vi "RemoteVI Landing Server.vi"(0 "VI":refnum<vi>, 1 "share":T1, 5 "port":u16=8088, 7 "fps":dbl=20.0, 9 "stop notifier name":string, 11 "error in":errorcluster) -> (15 "error out":errorcluster)   [LabVIEW 2020, in "RemoteVI.lvlib"]
doc: "RemoteVI Server's landing page: a small HTTP server on port that answers GET / (and /index.html) with the list of the shares of this application instance as links (RemoteVI Landing Page.vi from RemoteVI Status.vi) - but only with share.token as t= in the query (RemoteVI Token Check.vi), else 403; anything else 404; one request per connection, with the security headers (RemoteVI Send Static Response.vi). Listens at share's net address (127.0.0.1 = this computer only, 0 = every interface). Launched like a server loop (RemoteVI Launch Server Loop.vi sets the same controls - VI and fps are not used - and waits for the listener result on <stop notifier name>:started, RemoteVI Announce Listener.vi); it ends when the notifier stop notifier name delivers anything (RemoteVI Stop.vi with the same port)."
uses:
  RemoteVI.lvlib
  <vilib>/IlluminatedG/IG HTTP Utils/HTTP Utils/Request/Request.lvclass
  <vilib>/IlluminatedG/lv-stream/URI/URI.lvclass
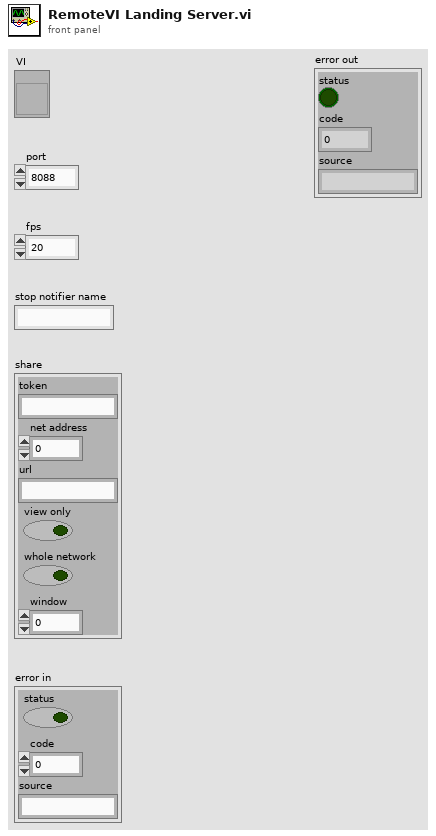
[diagram p1: front panel]
types:
  T1 = cluster{"token":string, "net address":u32, "url":string, "view only":bool, "whole network":bool, "window":u64}
  T2 = enum16{"standard", "buffered", "CRLF", "immediate"}
  T3 = cluster{"port":u16, "url":string, "target":string, "kind":string, "whole network":bool, "running":bool, "uptime s":dbl, "clients":cluster{"address":string, "connected s":dbl, "idle s":dbl}[], "fps":dbl, "kB per s":dbl, "frames":u32, "latency ms":dbl, "view only":bool, "last error":string, "hWnd":u64}[]
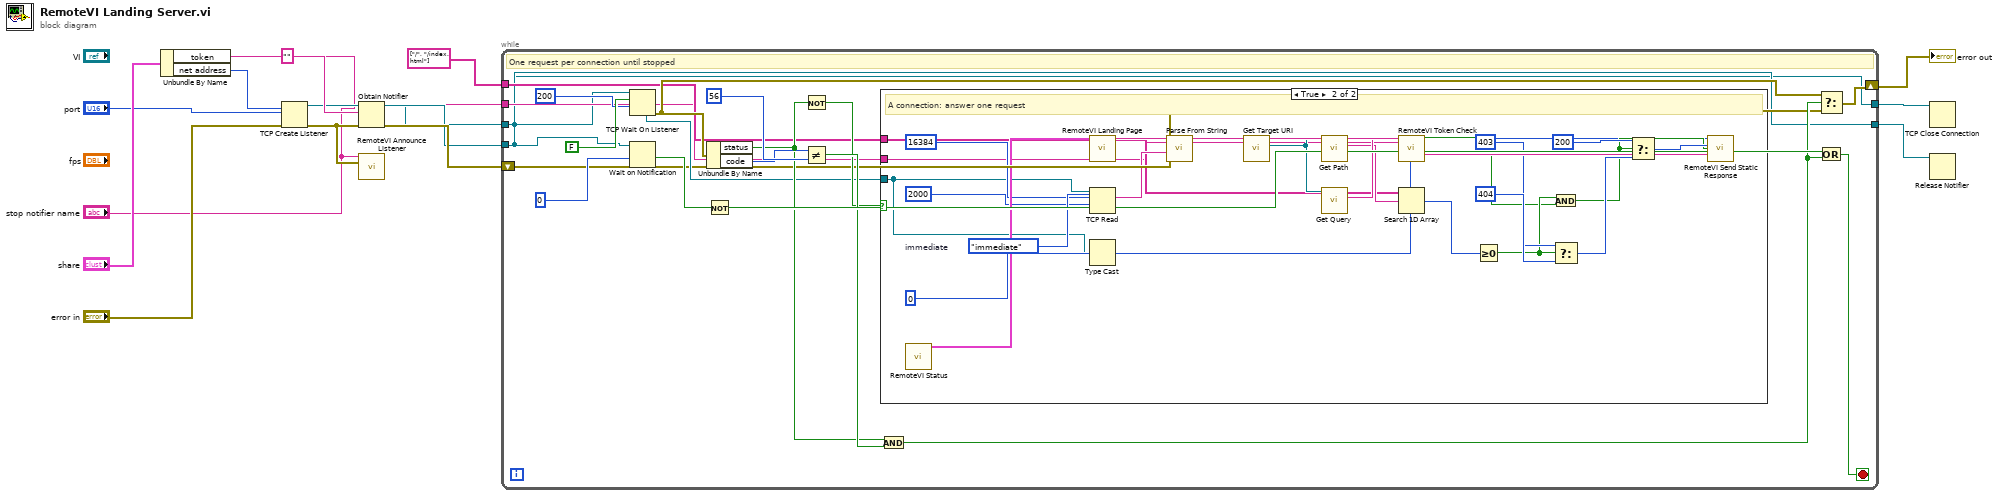
[diagram p0: block diagram]
diagram:
  n1 = Unbundle By Name("share") -> ("token"=w5:string, "net address"=w6:u32)
  n2 = TCP Create Listener(7:w6, 8:"error in", 10:"port") -> (0:w8:errorcluster, 3:w7:refnum<k5>)  [unwired: 2 in, 1 out]
  n3 = Obtain Notifier(name (unnamed)="stop notifier name", notification data type="", error in (no error)=w8) -> (notifier out=w10:refnum<notifier>, error out=w11:errorcluster)  [unwired: 1 in, 1 out]
  n4 = call "RemoteVI Announce Listener.vi"("stop notifier name"="stop notifier name", "listener result"=w8) -> ()  [unwired: 14 in]
  n5 = while {
    tunnel: string[] ["/", "/index.html"] -> [w19]
    tunnel: w5 -> [w18]
    tunnel: w7 -> [w16]
    tunnel: w10 -> [w17]
    shift-right: [w21] -> w13
    shift-left: w11 -> [w20]
    tunnel: [w16] -> w14
    tunnel: [w17] -> w15
    stop <- w35 stop-if-true
    # "One request per connection until stopped"
    n6 = TCP Wait On Listener(9:200, 10:FALSE, 11:w16) -> (0:w25:errorcluster, 4:w24:refnum<k5>)  [unwired: 1 in, 3 out]
    n7 = Wait on Notification(notifier=w17, timeout in ms (-1)=0) -> (timed out?=w33:bool)  [unwired: 2 in, 3 out]
    n8 = Unbundle By Name(w25) -> ("status"=w26:bool, "code"=w27:i32)
    n9 = Not(x=w33) -> (.not. x?=w34:bool)
    n10 = Not(x=w26) -> (.not. x?=w28:bool)
    n11 = Not Equal?(x=w27, y=56) -> (x != y?=w30:bool)
    n12 = case shown="True" w28 {
      tunnel: w19 -> [_ w38]
      tunnel: w18 -> [_ w37]
      tunnel: w24 -> [_ w36]
      frame False {
        # "No connection"
      }
      frame True {
        w41 = T2."immediate"  # immediate
        # "A connection: answer one request"
        n13 = call "RemoteVI Status.vi"() -> ("servers"=w58:T3)  [unwired: 14 in, 1 out]
        n14 = call "RemoteVI Landing Page.vi"("status"=w58) -> ("html"=w59:string)  [unwired: 14 in]
        n15 = TCP Read(connection ID=w36, bytes to read=16384, 7:w41, 9:2000) -> (data out=w42:string)  [unwired: 1 in, 2 out]
        n16 = Type Cast(type=u32 0, x=w36) -> (*(type *) &x=w44:u32)
        n17 = call <vilib>:"Parse From String.vi"("Request String"=w42) -> ("Request out"=w45:refnum<class "Request.lvclass">)  [unwired: 9 in, 1 out]
        n18 = call <vilib>:"Get Target URI.vi"("Request in"=w45) -> ("Target URI"=w46:refnum<class "URI.lvclass">)  [unwired: 8 in, 2 out]
        n19 = call <vilib>:"Get Path.vi"("URI in"=w46) -> ("Path"=w47:string)  [unwired: 8 in, 2 out]
        n20 = call <vilib>:"Get Query.vi"("URI in"=w46) -> ("Query"=w48:string)  [unwired: 8 in, 2 out]
        n21 = call "RemoteVI Token Check.vi"("query"=w48, "token"=w37) -> ("ok?"=w49:bool)  [unwired: 13 in]
        n22 = Search 1D Array(1D array=w38, element=w47) -> (index of element=w50:i32)  [unwired: 1 in]
        n23 = Greater Or Equal To 0?(x=w50) -> (x >= 0?=w51:bool)
        n24 = And(x=w51, y=w49) -> (x .and. y?=w52:bool)
        n25 = Select(t=u16 403, s=w51, f=u16 404) -> (s? t:f=w56:u16)
        n26 = Select(t=u16 200, s=w52, f=w56) -> (s? t:f=w57:u16)
        n27 = call "RemoteVI Send Static Response.vi"("connection"=w44, "status"=w57, "page?"=w52, "html"=w59) -> ()  [unwired: 11 in, 1 out]
      }
    }
    n28 = And(x=w26, y=w30) -> (x .and. y?=w31:bool)
    n29 = Select(t=w25, s=w31, f=w20) -> (s? t:f=w21:errorcluster)
    n30 = Or(x=w34, y=w31) -> (x .or. y?=w35:bool)
  }
  "error out" <- w13
  n31 = TCP Close Connection(connection ID=w14) -> ()  [unwired: 2 in, 2 out]
  n32 = Release Notifier(notifier=w15) -> ()  [unwired: 2 in, 3 out]
